vi "Test U8 Comm.vi"() -> ()   [LabVIEW 2021]
uses:
  <vilib>/CIF Foundation/CIF Channels Core/ChannelCommon/typedef/Direction.ctl
  <vilib>/CIF Foundation/CIF Channels Core/ChannelCommon/typedef/FIFO Config.ctl
  <vilib>/CIF Foundation/CIF Channels Core/ChannelCommon/typedef/TimeStamps.ctl
  CIF_CIPC_Fifo_U8.lvclass
  <vilib>/CIF Foundation/CIF Channels Core/ChannelCommon/ChannelCommon.lvlib
panel:
  out "status":string
  out "pass":bool
  out "error out":errorcluster
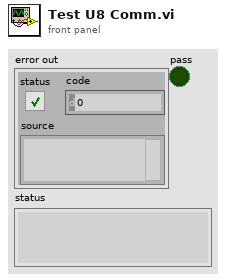
[diagram p1: front panel]
types:
  T1 = typedef "ChannelCommon.lvlib/Direction.ctl" = enum8{"Publisher", "Subscriber"}
  T2 = typedef "ChannelCommon.lvlib/TimeStamps.ctl" = cluster{"ClockID":u8, "T0":i64, "T_Out":i64}
  T3 = typedef "ChannelCommon.lvlib/FIFO Config.ctl" = cluster{"Max Bytes/Msg":u64, "Max Msg/FIFO":u64, "Flags":u64, "Custom Data":u8[]}
  T4 = typedef "ChannelCommon.lvlib/New FIFO Instance Response.ctl" = cluster{"Publisher":string, "Custom Data":u8[]}
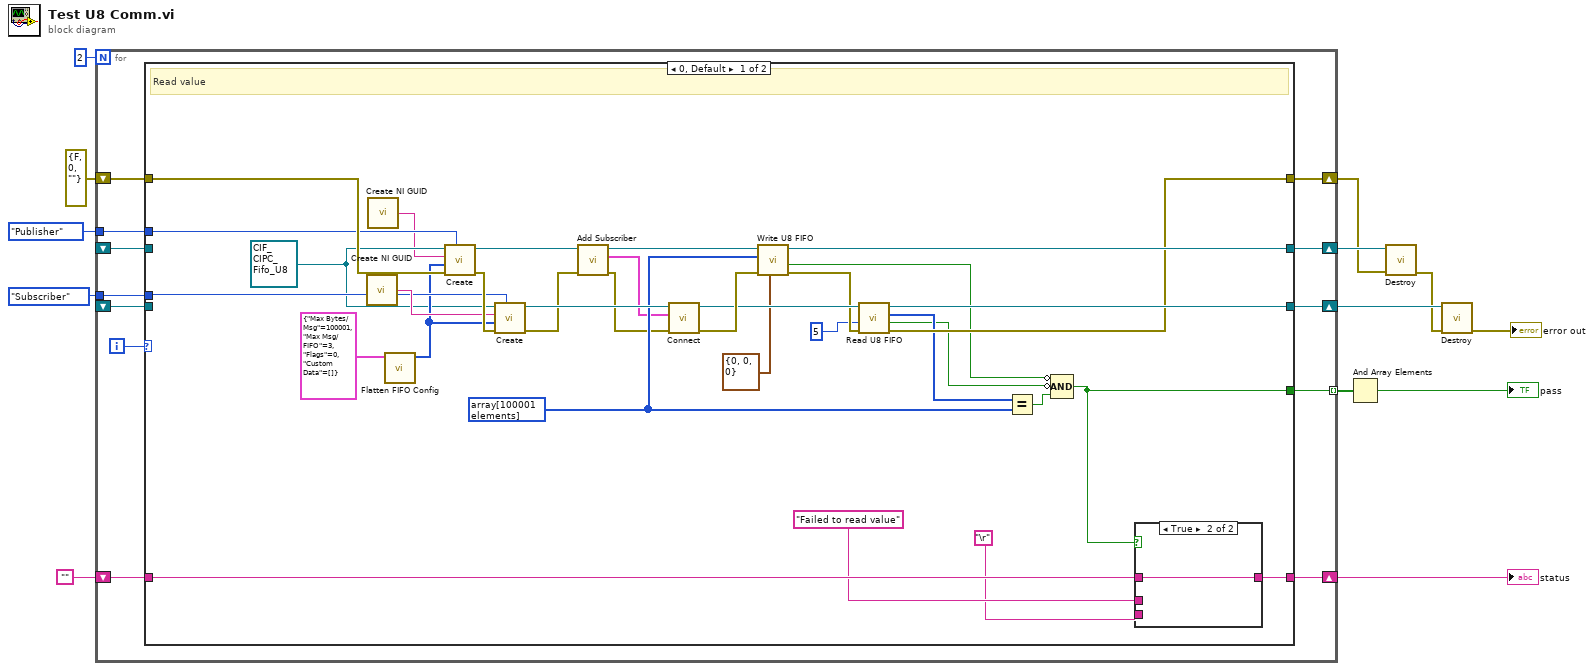
[diagram p0: block diagram]
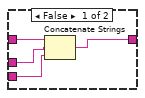
[diagram p2: hidden frame]
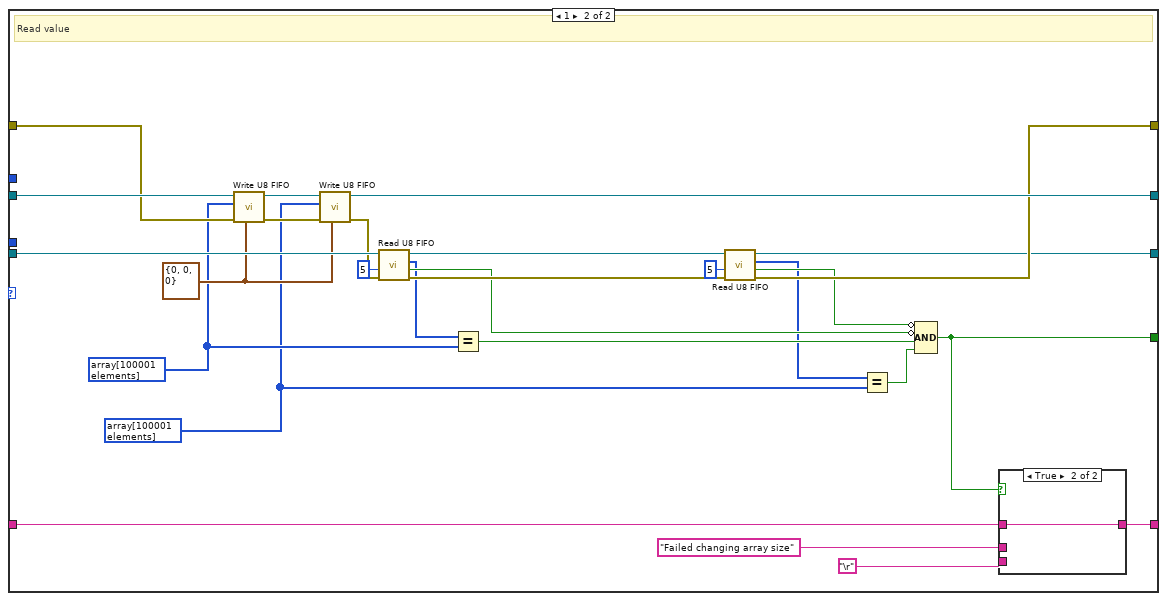
[diagram p3: hidden frame]
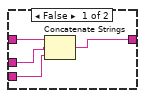
[diagram p4: hidden frame]
diagram:
  n1 = for {
    N: 2 -> [_]
    tunnel: [w25] -> w13 mode=indexing
    shift-right: [w23] -> w3
    shift-left: errorcluster {"status"=FALSE, "code"=0, "source"=""} ("error out") -> [w24]
    shift-right: [w20] -> w9
    shift-left: "" -> [w21]
    tunnel: Direction."Subscriber" ("Direction") -> [w19]
    tunnel: Direction."Publisher" ("Direction") -> [w18]
    shift-right: [w17] -> w5
    shift-left: _ -> [w15]
    shift-right: [w16] -> w4
    shift-left: _ -> [w14]
    i -> [w22]
    n2 = case shown="0, Default" w22 {
      tunnel: [w53 w86] -> w25
      tunnel: w24 -> [w51 w82]
      tunnel: [w41 w75] -> w23
      tunnel: w21 -> [w58 w90]
      tunnel: [w57 w89] -> w20
      tunnel: w19 -> [w49 _]
      tunnel: w18 -> [w48 _]
      tunnel: [w42 w72] -> w17
      tunnel: [w44 w79] -> w16
      tunnel: w14 -> [_ w83]
      tunnel: w15 -> [_ w78]
      frame 0, Default {
        w33 = refnum<class "CIF_CIPC_Fifo_U8.lvclass"> refnum ("CIF_CIPC_Fifo_U8.lvclass")
        w34 = u8[] array[100001 elements] ("U8 Data")
        # "Read value"
        n3 = call <vilib>:"Create NI GUID.vi"() -> ("NI GUID"=w50:string)
        n4 = call <vilib>:"Create NI GUID.vi"() -> ("NI GUID"=w29:string)
        n5 = call <vilib>:"Flatten FIFO Config.vi"("FIFO Config in"=T3 {"Max Bytes/Msg"=100001, "Max Msg/FIFO"=3, "Flags"=0, "Custom Data"=[]}) -> ("Flattened FIFO Config"=w35:u8[])  [unwired: 10 in]
        n6 = call-dynamic "Create.vi"("Direction"=w48, "error in (no error)"=w51, "Custom Config Data"=w35, "Name"=w29, "CIFFIFO in"=w33) -> ("error out"=w52:errorcluster, "CIFFIFO out"=w31:refnum<class "CIF_CIPC_Fifo_U8.lvclass">)  [unwired: 5 in]
        n7 = call-dynamic "Create.vi"("Direction"=w49, "error in (no error)"=w52, "Custom Config Data"=w35, "Name"=w50, "CIFFIFO in"=w33) -> ("error out"=w27:errorcluster, "CIFFIFO out"=w46:refnum<class "CIF_CIPC_Fifo_U8.lvclass">)  [unwired: 5 in]
        n8 = call-dynamic "Add Subscriber.vi"("error in (no error)"=w27, "CIF_CIPC_Chn in"=w31) -> ("error out"=w26:errorcluster, "New FIFO Instance"=w28:T4, "CIF_CIPC_Chn out"=w30:refnum<class "CIF_CIPC_Fifo_U8.lvclass">)  [unwired: 7 in]
        n9 = call-dynamic "Connect.vi"("error in (no error)"=w26, "Connection"=w28, "CIFTag in"=w46) -> ("error out"=w45:errorcluster, "CIFTag out"=w43:refnum<class "CIF_CIPC_Fifo_U8.lvclass">)  [unwired: 7 in]
        n10 = call-dynamic "Write U8 FIFO.vi"("FIFO Timestamps"=T2 {"ClockID"=0, "T0"=0, "T_Out"=0}, "error in (no error)"=w45, "Data in"=w34, "CIFFIFO in"=w30) -> ("error out"=w40:errorcluster, "timed out?"=w39:bool, "CIFFIFO out"=w44:refnum<class "CIF_CIPC_Fifo_U8.lvclass">)  [unwired: 4 in, 1 out]
        n11 = call-dynamic "Read U8 FIFO.vi"("error in (no error)"=w40, "Timeout (ms)"=5, "CIFFIFO in"=w43) -> ("error out"=w41:errorcluster, "timed out?"=w37:bool, "Data out"=w38:u8[], "CIFFIFO out"=w42:refnum<class "CIF_CIPC_Fifo_U8.lvclass">)  [unwired: 4 in, 1 out]
        n12 = Equal?(x=w38, y=w34) -> (x = y?=w54:bool)
        n13 = Compound Arithmetic op=AND(invert w39, invert w37, w54) -> (w53:bool)
        n14 = case shown="True" w53 {
          tunnel: w58 -> [w62 w63]
          tunnel: [w59 w63] -> w57
          tunnel: "Failed to read value" -> [w61 _]
          tunnel: "\r" -> [w60 _]
          frame False {
            n15 = Concatenate Strings(w62, w61, w60) -> (w59:string)
          }
          frame True {
          }
        }
      }
      frame 1 {
        w64 = u8[] array[100001 elements] ("U8 Data")
        w65 = u8[] array[100001 elements] ("U8 Data")
        w66 = T2 {"ClockID"=0, "T0"=0, "T_Out"=0} ("FIFO Timestamps")
        # "Read value"
        n16 = call-dynamic "Write U8 FIFO.vi"("FIFO Timestamps"=w66, "error in (no error)"=w82, "Data in"=w65, "CIFFIFO in"=w83) -> ("error out"=w80:errorcluster, "CIFFIFO out"=w81:refnum<class "CIF_CIPC_Fifo_U8.lvclass">)  [unwired: 4 in, 2 out]
        n17 = call-dynamic "Write U8 FIFO.vi"("FIFO Timestamps"=w66, "error in (no error)"=w80, "Data in"=w64, "CIFFIFO in"=w81) -> ("error out"=w76:errorcluster, "CIFFIFO out"=w79:refnum<class "CIF_CIPC_Fifo_U8.lvclass">)  [unwired: 4 in, 2 out]
        n18 = call-dynamic "Read U8 FIFO.vi"("error in (no error)"=w76, "Timeout (ms)"=5, "CIFFIFO in"=w78) -> ("error out"=w74:errorcluster, "timed out?"=w70:bool, "Data out"=w67:u8[], "CIFFIFO out"=w71:refnum<class "CIF_CIPC_Fifo_U8.lvclass">)  [unwired: 4 in, 1 out]
        n19 = Equal?(x=w67, y=w65) -> (x = y?=w84:bool)
        n20 = call-dynamic "Read U8 FIFO.vi"("error in (no error)"=w74, "Timeout (ms)"=5, "CIFFIFO in"=w71) -> ("error out"=w75:errorcluster, "timed out?"=w69:bool, "Data out"=w68:u8[], "CIFFIFO out"=w72:refnum<class "CIF_CIPC_Fifo_U8.lvclass">)  [unwired: 4 in, 1 out]
        n21 = Equal?(x=w68, y=w64) -> (x = y?=w85:bool)
        n22 = Compound Arithmetic op=AND(invert w69, invert w70, w84, w85) -> (w86:bool)
        n23 = case shown="True" w86 {
          tunnel: w90 -> [w94 w95]
          tunnel: [w91 w95] -> w89
          tunnel: "Failed changing array size" -> [w93 _]
          tunnel: "\r" -> [w92 _]
          frame False {
            n24 = Concatenate Strings(w94, w93, w92) -> (w91:string)
          }
          frame True {
          }
        }
      }
    }
  }
  "status" <- w9
  n25 = And Array Elements(Boolean array=w13) -> (logical AND=→"pass":bool)
  n26 = call-dynamic "Destroy.vi"("error in (no error)"=w3, "CIFTag in"=w4) -> ("error out"=w2:errorcluster)  [unwired: 8 in, 1 out]
  n27 = call-dynamic "Destroy.vi"("error in (no error)"=w2, "CIFTag in"=w5) -> ("error out"=→"error out":errorcluster)  [unwired: 8 in, 1 out]
